vi "VIH Utility - STR - Match Pattern - Find First Pattern.vi"(6 "offset (0)":i32, 8 "Regular expressions":string[](array[string]), 9 "String":string) -> (0 "offset past match":i32, 1 "after substring":string, 2 "match substring":string, 3 "before substring":string, 4 "first match index":i32)   [LabVIEW 2014]
doc: "::: VI Helpeks :::\nCopyright (c) 2000-2026 Konstantin Shifershteyn. All rights reserved."
panel:
  # "VI Helpeks\nCopyright (c) 2012-2026 Konstantin Shifershteyn"
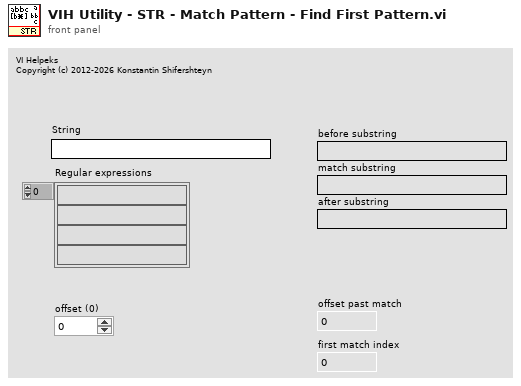
[diagram p1: front panel]
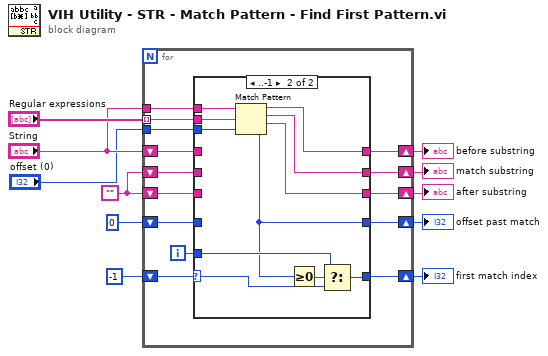
[diagram p0: block diagram]
diagram:
  w8 = ""
  n1 = for {
    shift-right: [w22] -> w10
    shift-left: -1 -> [w23]
    tunnel: "String" -> [w25]
    tunnel: "Regular expressions" -> [w24] mode=indexing
    shift-right: [w20] -> w5
    shift-left: "String" -> [w16]
    shift-right: [w19] -> w4
    shift-left: w8 -> [w15]
    shift-right: [w18] -> w3
    shift-left: w8 -> [w14]
    shift-right: [w17] -> w6
    shift-left: 0 ("offset past match") -> [w13]
    tunnel: "offset (0)" -> [w12]
    i -> [w21]
    n2 = case shown="..-1" w23 {
      selector: w23 -> [w30 w37]
      tunnel: w25 -> [_ w41]
      tunnel: w24 -> [_ w40]
      tunnel: [w30 w38] -> w22
      tunnel: w21 -> [_ w36]
      tunnel: [w29 w35] -> w20
      tunnel: [w28 w34] -> w19
      tunnel: [w27 w33] -> w18
      tunnel: [w26 w32] -> w17
      tunnel: w16 -> [w29 _]
      tunnel: w15 -> [w28 _]
      tunnel: w14 -> [w27 _]
      tunnel: w13 -> [w26 _]
      tunnel: w12 -> [_ w31]
      frame 0.. {
      }
      frame ..-1 {
        n3 = Match Pattern(string=w41, regular expression=w40, offset (0)=w31) -> (before substring=w35:string, match substring=w34:string, after substring=w33:string, offset past match=w32:i32)
        n4 = Greater Or Equal To 0?(x=w32) -> (x >= 0?=w39:bool)
        n5 = Select(t=w36, s=w39, f=w37) -> (s? t:f=w38:i32)
      }
    }
  }
  "first match index" <- w10
  "offset past match" <- w6
  "before substring" <- w5
  "match substring" <- w4
  "after substring" <- w3
